vi "Initialize 8 NEO Swerve Drive.vi"() -> (0 "error out":errorcluster, 3 "(N-N-C-P) Swerve Motors":T1 {"Steer Scaling" format="%.2f"; "Drive Scaling" format="%.2f"; "Pod Locations (ft)"."Right Back Position" format="%.2f"; "Pod Locations (ft)"."Right Front Position" format="%.2f"; "Pod Locations (ft)"."Left Back Position" format="%.2f"; "Pod Locations (ft)"."Left Front Position" format="%.2f"})   [LabVIEW 2027]
doc: "Creates a cluster of 4 motors (order is left-front, left-back, right-front, right-back) initialized with PID coefficients and status frame reduction"
uses:
  Type Definitions/Hardware/Swerve Drives/(NEO-NEO-ThroughBore-Pigeon2) Swerve.ctl
  <vilib>/REV Custom Controls/REVSparkRefnum.ctl
  Type Definitions/Data/Pod Positions.ctl
  Type Definitions/Hardware/Swerve Configs/NEO-NEO-ThroughBore-Pigeon2 Swerve Config.ctl
  <vilib>/REV Custom Controls/Spark Voltage Compensation.ctl
  <vilib>/REVLibDriver/REVLibDriver.lvlib
  <resource>/objmgr/REVSpark.rc
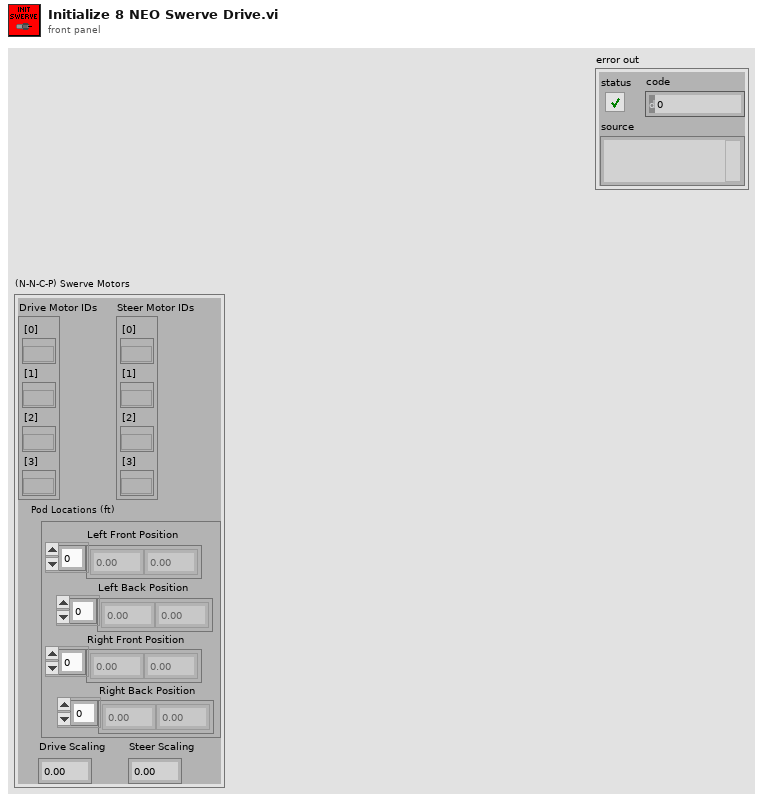
[diagram p1: front panel]
types:
  T1 = typedef "(NEO-NEO-ThroughBore-Pigeon2) Swerve.ctl" = cluster{"Drive Motor IDs":cluster{"[0]":T2, "[1]":T2, "[2]":T2, "[3]":T2}, "Steer Motor IDs":cluster{"[0]":T2, "[1]":T2, "[2]":T2, "[3]":T2}, "Pod Locations (ft)":T3, "Drive Scaling":dbl, "Steer Scaling":dbl}
  T2 = typedef "REVLibDriver.lvlib/REVSparkRefnum.ctl" = refnum<k20>
  T3 = typedef "Pod Positions.ctl" = cluster{"Left Front Position":dbl[], "Left Back Position":dbl[], "Right Front Position":dbl[], "Right Back Position":dbl[]}
  T4 = typedef "NEO-NEO-ThroughBore-Pigeon2 Swerve Config.ctl" = cluster{"Bus ID":dbl, "Drive Motor CAN IDs":cluster{"LF CAN ID":dbl, "LB CAN ID":dbl, "RF CAN ID":dbl, "RB CAN ID":dbl}, "Steer Motor CAN IDs":cluster{"LF CAN ID":dbl, "LB CAN ID":dbl, "RF CAN ID":dbl, "RB CAN ID":dbl}, "Drive PID Gains":cluster{cluster{"P Gain":dbl, "I Gain":dbl, "D Gain":dbl, "kV":dbl}, "I Zone":dbl, "Output LImits":cluster{"Min Output":dbl, "Max Output":dbl}}, "Steer PID Gains":cluster{cluster{"P Gain":dbl, "I Gain":dbl, "D Gain":dbl, "kV":dbl}, "I Zone":dbl, "Output LImits":cluster{"Min Output":dbl, "Max Output":dbl}}, "Pod Locations (ft)":T3, "Inverted":cluster{"LF Inverted?":bool, "LFBInverted":bool, "RF Inverted":bool, "RB Inverted":bool}}
  T5 = cluster{"LF CAN ID":dbl, "LB CAN ID":dbl, "RF CAN ID":dbl, "RB CAN ID":dbl}
  T6 = cluster{cluster{"P Gain":dbl, "I Gain":dbl, "D Gain":dbl, "kV":dbl}, "I Zone":dbl, "Output LImits":cluster{"Min Output":dbl, "Max Output":dbl}}
  T7 = typedef "REVLibDriver.lvlib/Spark Voltage Compensation.ctl" = cluster{"Mode":u32, "Nominal Voltage":dbl}
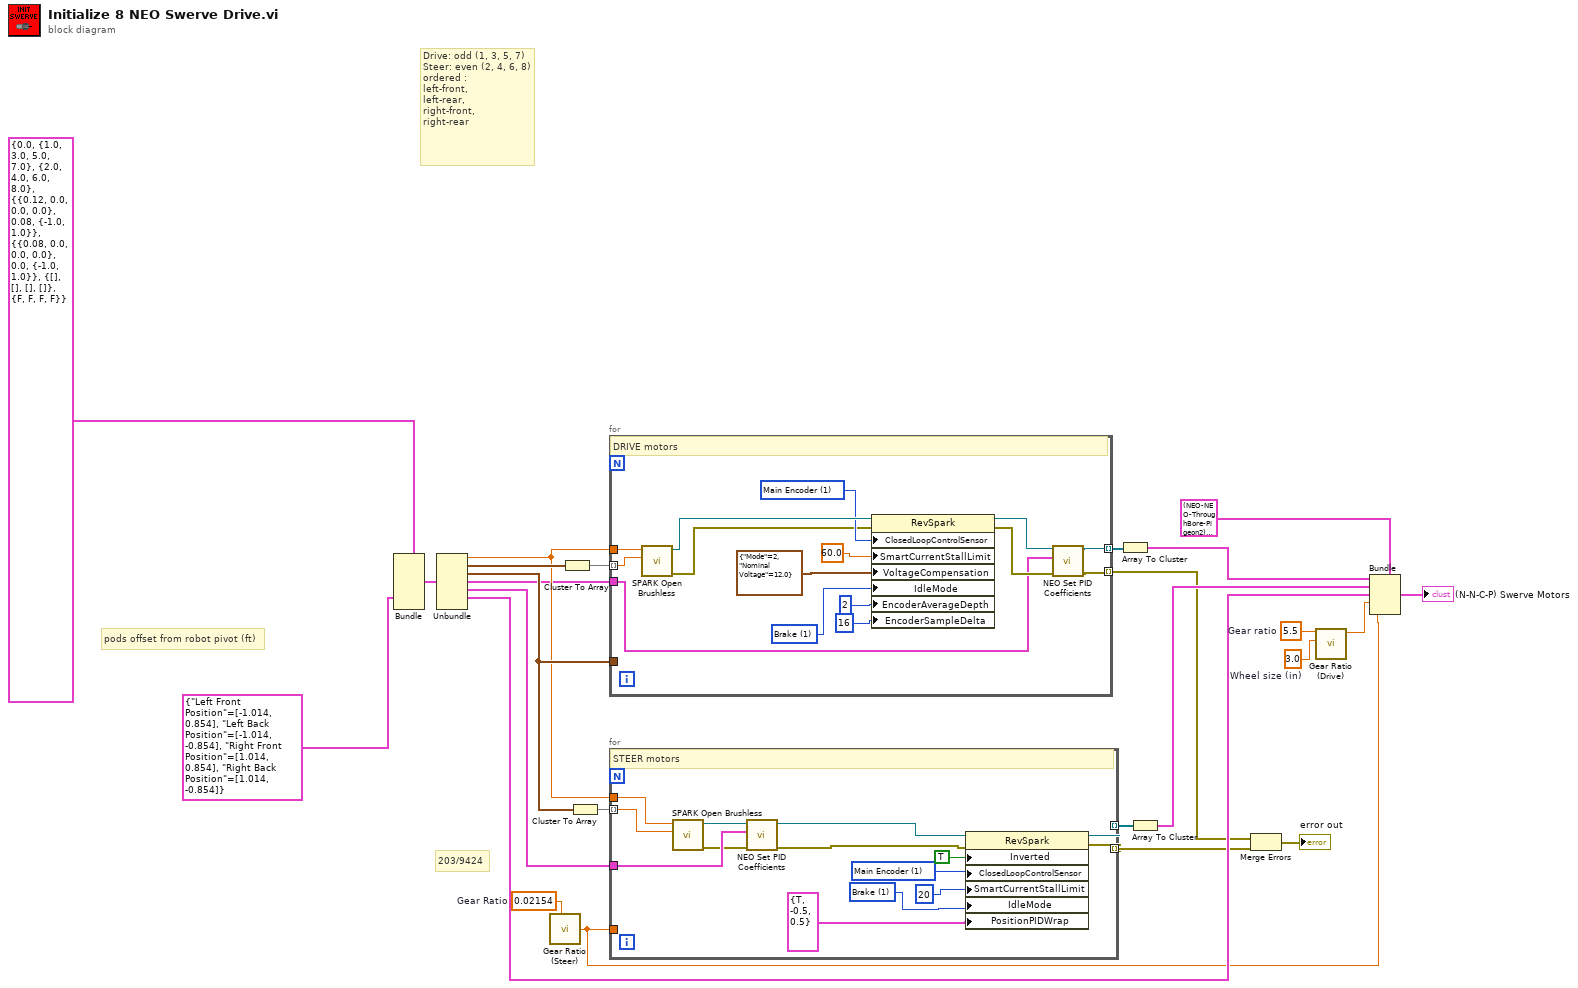
[diagram p0: block diagram]
diagram:
  w2 = 0.02154  # Gear Ratio
  w5 = 3.0  # Wheel size (in)
  w4 = 5.5  # Gear ratio
  # "203/9424"
  # "Drive: odd (1, 3, 5, 7)\nSteer: even (2, 4, 6, 8)\nordered :\nleft-front,\nleft-rear,\nright-front,\nright-rear"
  # "pods offset from robot pivot (ft)"
  n1 = Bundle(cluster=T4 {"Bus ID"=0.0, "Drive Motor CAN IDs"={"LF CAN ID"=1.0, "LB CAN ID"=3.0, "RF CAN ID"=5.0, "RB CAN ID"=7.0}, "Steer Motor CAN IDs"={"LF CAN ID"=2.0, "LB CAN ID"=4.0, "RF CAN ID"=6.0, "RB CAN ID"=8.0}, "Drive PID Gains"={{"P Gain"=0.12, "I Gain"=0.0, "D Gain"=0.0, "kV"=0.0}, "I Zone"=0.08, "Output LImits"={"Min Output"=-1.0, "Max Output"=1.0}}, "Steer PID Gains"={{"P Gain"=0.08, "I Gain"=0.0, "D Gain"=0.0, "kV"=0.0}, "I Zone"=0.0, "Output LImits"={"Min Output"=-1.0, "Max Output"=1.0}}, "Pod Locations (ft)"={"Left Front Position"=[], "Left Back Position"=[], "Right Front Position"=[], "Right Back Position"=[]}, "Inverted"={"LF Inverted?"=FALSE, "LFBInverted"=FALSE, "RF Inverted"=FALSE, "RB Inverted"=FALSE}} ("Swerve Config"), "Pod Locations (ft)"=T3 {"Left Front Position"=[-1.014, 0.854], "Left Back Position"=[-1.014, -0.854], "Right Front Position"=[1.014, 0.854], "Right Back Position"=[1.014, -0.854]} ("Radii (ft)")) -> (w23:T4)  [unwired: 6 in]
  n2 = Unbundle(w23) -> ("Bus ID"=w10:dbl, "Drive Motor CAN IDs"=w12:T5, "Steer Motor CAN IDs"=w11:T5, "Drive PID Gains"=w9:T6, "Steer PID Gains"=w8:T6, "Pod Locations (ft)"=w21:T3)  [unwired: 1 out]
  n3 = call "Gear Ratio (Steer).vi"("Gear Ratio"=w2) -> ("Position Factor"=w1:dbl)  [unwired: 6 in, 1 out]
  n4 = Cluster To Array(cluster=w12) -> (array=w25:dbl[])
  n5 = Cluster To Array(cluster=w11) -> (array=w24:dbl[])
  n6 = for {
    tunnel: w25 -> [w40] mode=indexing
    tunnel: w11 -> [_]
    tunnel: [w27] -> w19 mode=indexing
    tunnel: [w26] -> w15 mode=indexing
    tunnel: w10 -> [w39]
    tunnel: w9 -> [w33]
    w30 = u32 1 items=["Coast", "Brake"] ("IdleMode")
    w37 = u32 1 items=["None", "Main Encoder", "Analog", "Alt Encoder", "Duty Cycle", "Detached Absolute", "Detached Relative"] ("ClosedLoopControlSensor")
    # "DRIVE motors"
    n7 = call <vilib>:"SPARK Open Brushless.vi"("deviceId"=w40, "busID"=w39) -> ("error out"=w35:errorcluster, "Spark refnum"=w38:T2)  [unwired: 8 in]
    n8 = property class="RevSpark"(reference=w38, error in=w35, "ClosedLoopControlSensor"=w37, "SmartCurrentStallLimit"=60.0 ("Primay Current Limit (80A)"), "VoltageCompensation"=T7 {"Mode"=2, "Nominal Voltage"=12.0}, "IdleMode"=w30, "EncoderAverageDepth"=u32 2, "EncoderSampleDelta"=u32 16) -> (reference out=w36:T2, error out=w34:errorcluster)
    n9 = call "NEO Set PID Coefficients.vi"("error in"=w34, "PID Gains"=w33, "Spark refnum"=w36) -> ("error out"=w26:errorcluster, "Spark refnum out"=w27:T2)  [unwired: 5 in]
  }
  n10 = for {
    tunnel: w24 -> [w53] mode=indexing
    tunnel: w8 -> [w54]
    tunnel: [w45] -> w17 mode=indexing
    tunnel: [w43] -> w16 mode=indexing
    tunnel: w10 -> [w52]
    tunnel: w1 -> [_]
    w49 = u32 1 items=["None", "Main Encoder", "Analog", "Alt Encoder", "Duty Cycle", "Detached Absolute", "Detached Relative"] ("ClosedLoopControlSensor")
    w47 = u32 1 items=["Coast", "Brake"] ("IdleMode")
    # "STEER motors"
    n11 = call <vilib>:"SPARK Open Brushless.vi"("deviceId"=w53, "busID"=w52) -> ("error out"=w50:errorcluster, "Spark refnum"=w51:T2)  [unwired: 8 in]
    n12 = call "NEO Set PID Coefficients.vi"("error in"=w50, "PID Gains"=w54, "Spark refnum"=w51) -> ("error out"=w44:errorcluster, "Spark refnum out"=w46:T2)  [unwired: 5 in]
    n13 = property class="RevSpark"(reference=w46, error in=w44, "Inverted"=TRUE ("Invert"), "ClosedLoopControlSensor"=w49, "SmartCurrentStallLimit"=u32 20, "IdleMode"=w47, "PositionPIDWrap"=cluster{"Enable":bool, "Min":sgl, "Max":sgl} {"Enable"=TRUE, "Min"=-0.5, "Max"=0.5}) -> (reference out=w45:T2, error out=w43:errorcluster)
  }
  n14 = Array To Cluster(array=w19) -> (cluster=w14:cluster{"[0]":T2, "[1]":T2, "[2]":T2, "[3]":T2})
  n15 = Array To Cluster(array=w17) -> (cluster=w18:cluster{"[0]":T2, "[1]":T2, "[2]":T2, "[3]":T2})
  n16 = Merge Errors(w15, w16) -> (→"error out":errorcluster)
  n17 = call "Gear Ratio (Drive).vi"("Wheel size (in)"=w5, "Gear ratio"=w4) -> ("Velocity Factor (ft/s)"=w3:dbl)  [unwired: 9 in]
  n18 = Bundle(cluster=T1 {"Drive Motor IDs"={"[0]"=refnum, "[1]"=refnum, "[2]"=refnum, "[3]"=refnum}, "Steer Motor IDs"={"[0]"=refnum, "[1]"=refnum, "[2]"=refnum, "[3]"=refnum}, "Pod Locations (ft)"={"Left Front Position"=[], "Left Back Position"=[], "Right Front Position"=[], "Right Back Position"=[]}, "Drive Scaling"=0.0, "Steer Scaling"=0.0} ("(N-N-C-P) Swerve Motors"), "Drive Motor IDs"=w14, "Steer Motor IDs"=w18, "Pod Locations (ft)"=w21, "Drive Scaling"=w3, "Steer Scaling"=w1) -> (→"(N-N-C-P) Swerve Motors":T1)
